vi "ReversedEngineering_GetClassPathFromNode.vi"(0 "reference":refnum<class "AbstractNode.lvclass">, 5 "error IO":errorcluster) -> (15 "Path":path, 19 "error out":errorcluster)   [LabVIEW 2020]
uses:
  <resource>/Framework/Providers/Open_GDS/UML/AbstractNode_class/AbstractNode.lvclass
  <resource>/Framework/Providers/Open_GDS/UML/ClassNode_class/ExternalSetTypes.ctl
  <resource>/Framework/Providers/Open_GDS/UML/ClassNode_class/ClassNode.lvclass
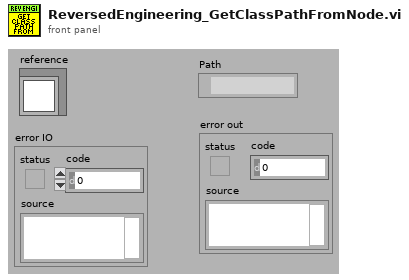
[diagram p1: front panel]
types:
  T1 = typedef "ClassNode.lvclass/ExternalSetTypes.ctl" = enum16{"Name", "Attributes", "Methods", "Position", "ShowMethods", "ShowAttributes", "ClassPath"}
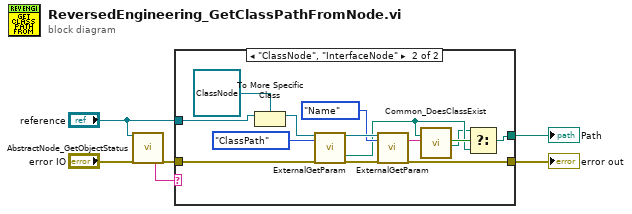
[diagram p0: block diagram]
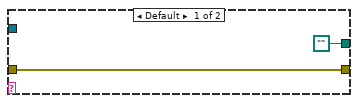
[diagram p2: hidden frame]
diagram:
  n1 = call <resource>:"AbstractNode_GetObjectStatus.vi"("reference in"="reference", "error in (no error)"="error IO") -> ("Class name"=w1:string, "error out"=w6:errorcluster)  [unwired: 16 out]
  n2 = case shown="\"ClassNode\", \"InterfaceNode\"" w1 {
    tunnel: "reference" -> [_ w11]
    tunnel: w6 -> [w8 w12]
    tunnel: [w8 w17] -> w2
    tunnel: [path "" w13] -> w3
    frame Default {
    }
    frame "ClassNode", "InterfaceNode" {
      n3 = To More Specific Class(target class=refnum<class "ClassNode.lvclass"> refnum ("reference"), reference=w11) -> (specific class reference=w9:refnum<class "ClassNode.lvclass">)  [unwired: 1 in, 1 out]
      n4 = call <resource>:"ExternalGetParam.vi"("reference"=w9, "setParameter"=ExternalSetTypes."ClassPath", "error in (no error)"=w12) -> ("reference out"=w21:refnum<class "ClassNode.lvclass">, "Path"=w15:path, "error out"=w20:errorcluster)  [unwired: 14 out]
      n5 = call <resource>:"ExternalGetParam.vi"("reference"=w21, "setParameter"=ExternalSetTypes."Name", "error in (no error)"=w20) -> ("string"=w18:string, "error out"=w17:errorcluster)  [unwired: 15 out]
      n6 = call <resource>:"Common_DoesClassExist.vi"("ClassPath"=w15, "ClassName"=w18) -> ("llb-class"=w16:bool, "llb/LvCLass-Path"=w14:path)  [unwired: 16 out]
      n7 = Select(t=w14, s=w16, f=w15) -> (s? t:f=w13:path)
    }
  }
  "Path" <- w3
  "error out" <- w2
